vi "Initialise TCP.vi"(6 "Tag Root":string, 8 "error in (no error)":errorcluster, 9 "Channels":refnum<class "Abs_Value.lvclass">[](array[class]), 10 "VISA resource name":refnum<visa-resource-name>, 11 "CTI_TCP_Bus in":refnum<class "CTI_TCP_Bus.lvclass">) -> (0 "error out":errorcluster, 3 "CTI_TCP_Bus out":refnum<class "CTI_TCP_Bus.lvclass">)   [LabVIEW 2021, in "CTI_TCP_Bus.lvclass"]
uses:
  CTI_TCP_Bus.lvclass
  C:/TSA/CTI-Bus/Source/Parent/CTI_Bus.lvclass
  C:/Program Files (x86)/National Instruments/LabVIEW 2021/vi.lib/TSA/Omni-Bus/Omni-Bus/Bus Access/Bus_Access.lvclass
  <vilib>/TSA/Abstract Data Classes/Abs_Types/Value/Abs_Value.lvclass
  C:/Program Files (x86)/National Instruments/LabVIEW 2021/vi.lib/TSA/Abstract Data Classes/Abs_Types/Type/Abs_Type.lvclass
  Parent/CTI_Bus.lvclass/CTI_Bus.ctl
  <vilib>/TSA/Omni-Bus/Omni-Bus/Bus Access/Bus_Access.lvclass/Bus_Access.ctl
  Parent/Properties/Write VISA resource name.vi
  Parent/Properties/Write Channels.vi
  <vilib>/TSA/Omni-Bus/Omni-Bus/Bus Access/Properties/Write Tag Root.vi
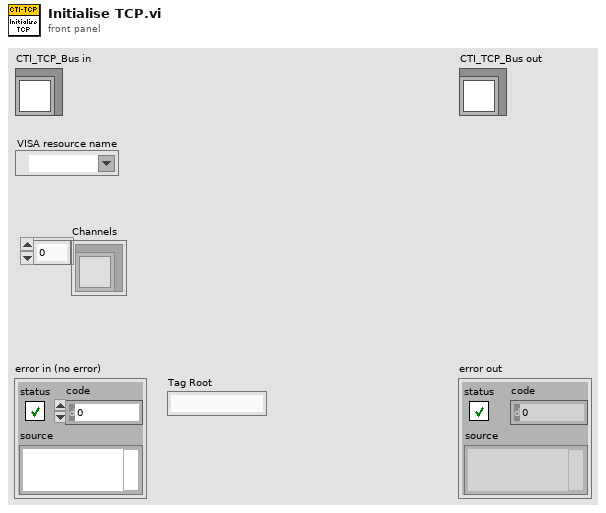
[diagram p1: front panel]
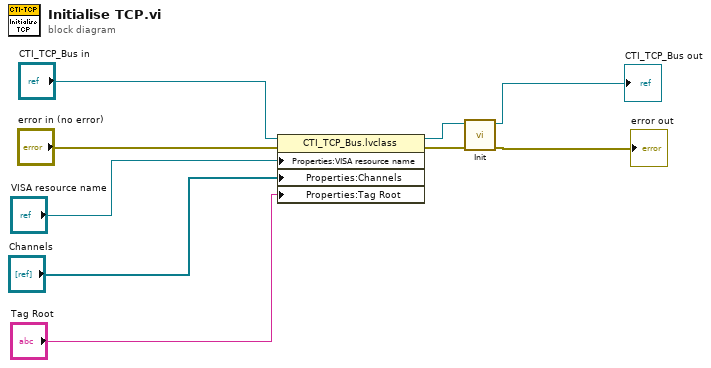
[diagram p0: block diagram]
diagram:
  n1 = property class="CTI_TCP_Bus.lvclass"(reference="CTI_TCP_Bus in", error in="error in (no error)", "Properties:VISA resource name"="VISA resource name", "Properties:Channels"="Channels", "Properties:Tag Root"="Tag Root") -> (reference out=w7:refnum<class "CTI_TCP_Bus.lvclass">, error out=w8:errorcluster)
  n2 = call-dynamic "Init.vi"("error in (no error)"=w8, "Data in"=w7) -> ("error out"=→"error out":errorcluster, "Data out"=→"CTI_TCP_Bus out":refnum<class "CTI_TCP_Bus.lvclass">)  [unwired: 8 in]
